vi "VIH HelpGen - Palette - Read Palette (non-palette allowed).vi"(7 "Get Items (F)":bool, 8 "error in":errorcluster, 10 "palette type":T1=-1 items=["Functions"=-1, "Controls"=-2], 11 "Palette Path":path) -> (0 "error out":errorcluster, 1 "palette data":T2={"display name"="", "view format"=0, "palette width"=4, "items"=[], "256 color icon"=bytes[0], "B&W color icon"=bytes[0], "help information"={"help tag"="", "help file path "=path ""}, "palette description"="", "synchronize information"={"synchronize with directory"=FALSE, "synchronize directory path"=path ""}} {"view format" items=["Icons", "Text", "Icons and Text"]}, 3 "dup Palette Menu Path":path)   [LabVIEW 2014]
doc: "::: VI Helpeks :::\nCopyright (c) 2000-2026 Konstantin Shifershteyn. All rights reserved."
uses:
  <vilib>/Palette API/Palette Menu/Public Type Define/Palette Data.ctl
  <vilib>/Palette API/Palette Menu/Public Type Define/View Format.ctl
  <vilib>/Palette API/Palette Menu/Public Type Define/Items.ctl
  <vilib>/Palette API/Palette Menu/Public Type Define/Item.ctl
  <vilib>/Palette API/Palette Menu/Public Type Define/Help Info.ctl
  <vilib>/Palette API/Palette Menu/Public Type Define/Synchronize Info.ctl
  <vilib>/Palette API/Palette Menu/Public Type Define/Palette type.ctl
  <vilib>/Palette API/Palette Menu/Palette Menu.lvlib
panel:
  in  "DefIcon - Default Palette":picture
  # "VI Helpeks\nCopyright (c) 2012-2026 Konstantin Shifershteyn"
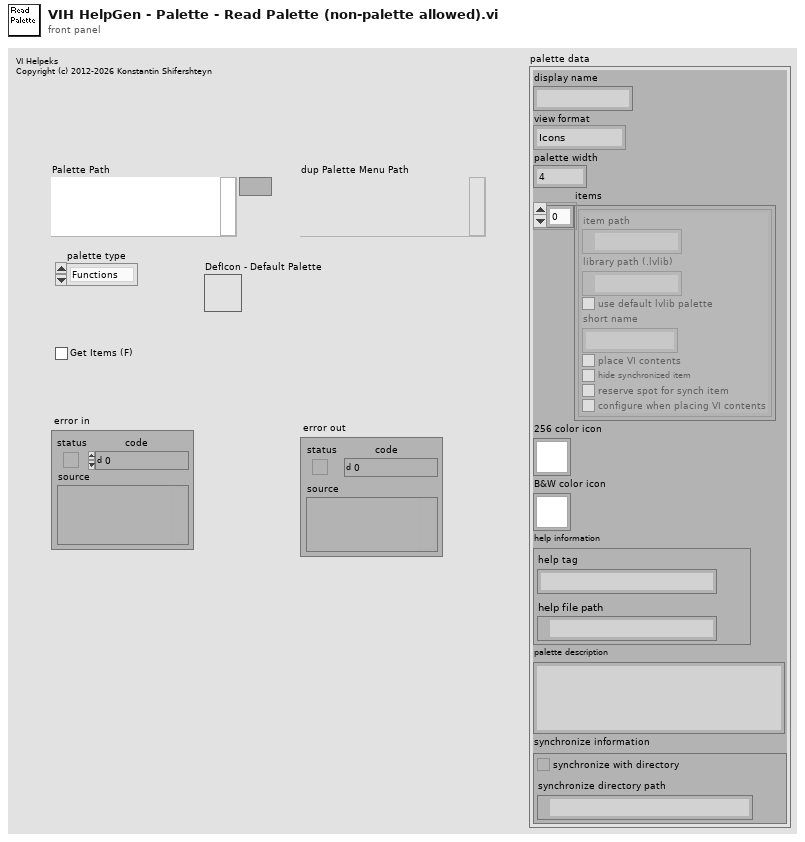
[diagram p1: front panel]
types:
  T1 = typedef "Palette Menu.lvlib/Palette type.ctl" = i32
  T2 = typedef "Palette Menu.lvlib/Palette Data.ctl" = cluster{"display name":string, "view format":T3, "palette width":i16, "items":T4, "256 color icon":picture, "B&W color icon":picture, "help information":T6, "palette description":string, "synchronize information":T7}
  T3 = typedef "Palette Menu.lvlib/View Format.ctl" = u16
  T4 = typedef "Palette Menu.lvlib/Items.ctl" = T5[]
  T5 = typedef "Palette Menu.lvlib/Item.ctl" = cluster{"item path":path, "library path (.lvlib)":path, "use default lvlib palette":bool, "short name":string, "place VI contents":bool, "hide synchronized item":bool, "reserve spot for synch item":bool, "configure when placing VI contents":bool}
  T6 = typedef "Palette Menu.lvlib/Help Info.ctl" = cluster{"help tag":string, "help file path ":path}
  T7 = typedef "Palette Menu.lvlib/Synchronize Info.ctl" = cluster{"synchronize with directory":bool, "synchronize directory path":path}
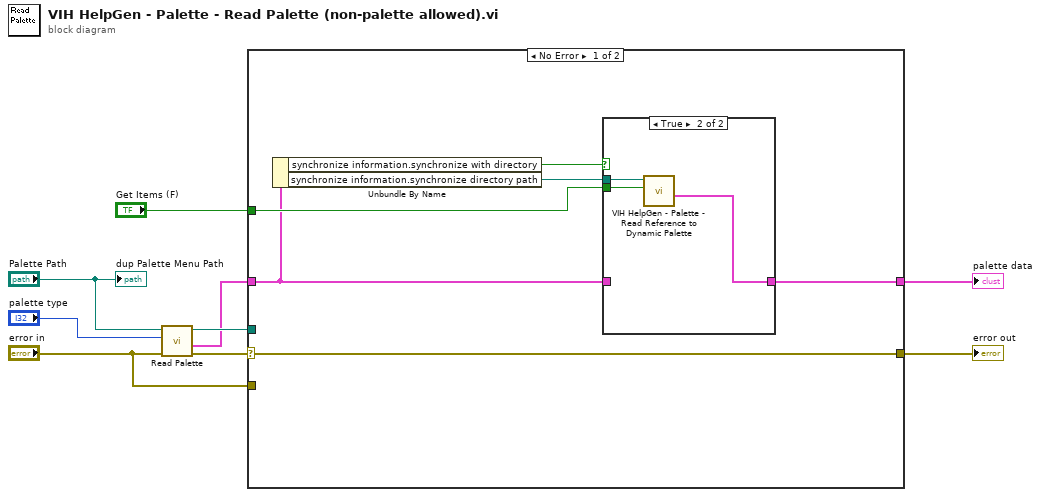
[diagram p0: block diagram]
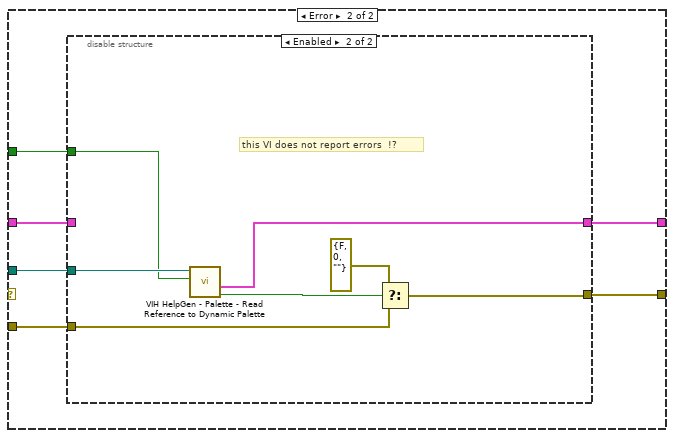
[diagram p3: hidden frame]
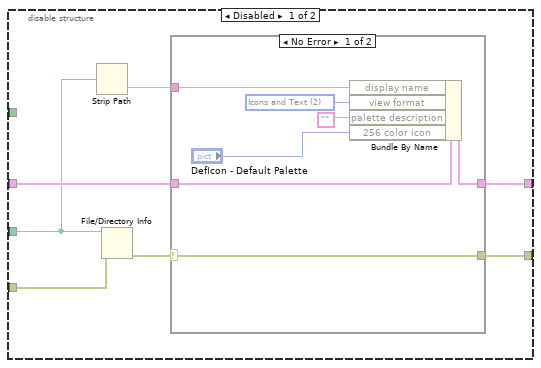
[diagram p4: hidden frame]
diagram:
  n1 = call <vilib>:"Read Palette.vi"("error in (no error)"="error in", "palette type"="palette type", "palette path"="Palette Path") -> ("error out"=w8:errorcluster, "palette data"=w4:T2, "duplicate palette path"=w7:path)  [unwired: 6 in]
  n2 = case shown="No Error" w8 {
    selector: w8 -> [w10 _]
    tunnel: w7 -> [_ w22]
    tunnel: [w10 w21] -> w6
    tunnel: "error in" -> [_ w25]
    tunnel: w4 -> [w11 w24]
    tunnel: [w12 w23] -> w3
    tunnel: "Get Items (F)" -> [w15 w20]
    frame No Error {
      n3 = Unbundle By Name(w11) -> ("synchronize information.synchronize with directory"=w13:bool, "synchronize information.synchronize directory path"=w14:path)
      n4 = case shown="True" w13 {
        tunnel: w14 -> [_ w19]
        tunnel: w15 -> [_ w18]
        tunnel: [w16 w17] -> w12
        tunnel: w11 -> [w16 _]
        frame False {
        }
        frame True {
          n5 = call "VIH HelpGen - Palette - Read Reference to Dynamic Palette.vi"("Get Items (F)"=w18, "Palette Path"=w19) -> ("palette data"=w17:T2)  [unwired: 8 in, 1 out]
        }
      }
    }
    frame Error {
      n6 = disable-structure shown="Enabled" {
        disable-tunnel: w25 -> [w32 w45]
        disable-tunnel: w24 -> [w31 _]
        disable-tunnel: [w30 w47] -> w23
        disable-tunnel: w22 -> [w28 w48]
        disable-tunnel: [w26 w44] -> w21
        disable-tunnel: w20 -> [_ w43]
        frame Disabled {
          n7 = Strip Path(path=w28) -> (name=w27:string)  [unwired: 1 out]
          n8 = File/Directory Info(path=w28, error in=w32) -> (error out=w29:errorcluster)  [unwired: 6 out]
          n9 = case shown="No Error" w29 {
            selector: w29 -> [w33 w40]
            tunnel: w31 -> [w39 w41]
            tunnel: [w36 w41] -> w30
            tunnel: w27 -> [w34 _]
            tunnel: [w33 w40] -> w26
            frame No Error {
              w38 = T3 2 items=["Icons", "Text", "Icons and Text"] ("view format")
              n10 = Bundle By Name(cluster=w39, "display name"=w34, "view format"=w38, "palette description"="", "256 color icon"="DefIcon - Default Palette") -> (w36:T2)
            }
            frame Error {
            }
          }
        }
        frame Enabled {
          # "this VI does not report errors  !?"
          n11 = call "VIH HelpGen - Palette - Read Reference to Dynamic Palette.vi"("Get Items (F)"=w43, "Palette Path"=w48) -> ("Data available"=w46:bool, "palette data"=w47:T2)  [unwired: 8 in]
          n12 = Select(t=errorcluster {"status"=FALSE, "code"=0, "source"=""}, s=w46, f=w45) -> (s? t:f=w44:errorcluster)
        }
      }
    }
  }
  "error out" <- w6
  "palette data" <- w3
  "dup Palette Menu Path" <- "Palette Path"
